vi "TurretAim_OperatorAssist.vi"(0 "Reacquire":bool, 1 "Start":bool, 2 "ManualOverride":bool, 3 "TargetFound":bool, 4 "FullRight":bool, 5 "FullLeft":bool, 8 "TargetPos":dbl format="%#_13g") -> (6 "TurretPos":dbl format="%#_13g", 7 "Current_State":T1=enum."SearchLeft")   [LabVIEW 2016]
uses:
  TypeDefs/TurretAimState_Type.ctl
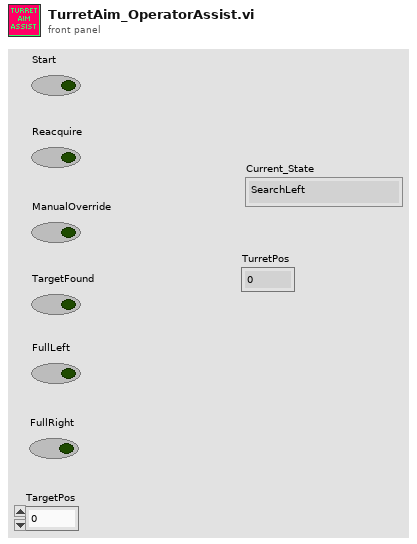
[diagram p1: front panel]
types:
  T1 = typedef "TurretAimState_Type.ctl" = enum16{"Idle", "SearchLeft", "SearchRight", "FindNewTarget", "TargetAcquired"}
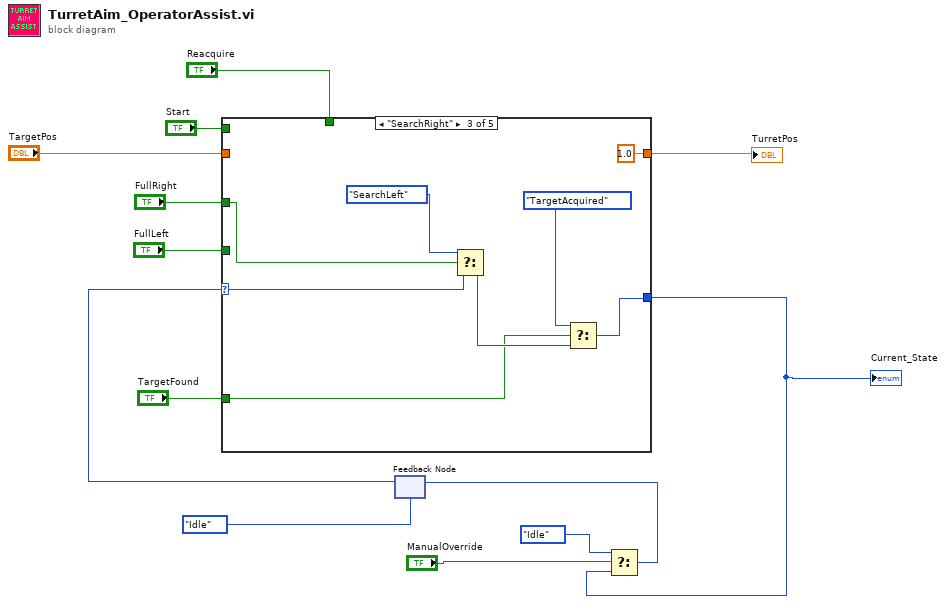
[diagram p0: block diagram]
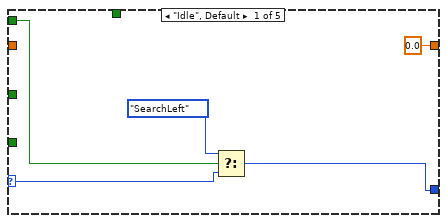
[diagram p2: hidden frame]
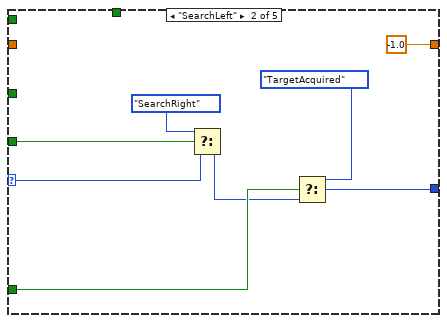
[diagram p3: hidden frame]
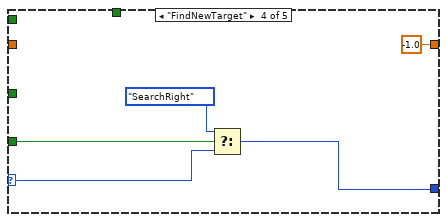
[diagram p4: hidden frame]
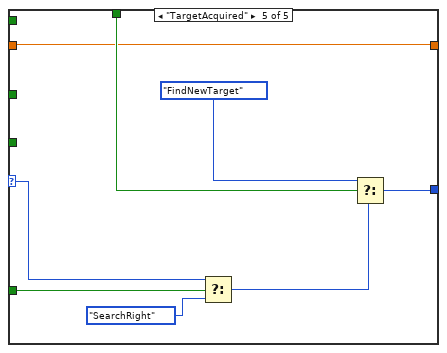
[diagram p5: hidden frame]
diagram:
  n1 = feedback #1(TurretAimState_Type."Idle" ("TurretState")) -> (w13:T1)
  n2 = case shown="\"SearchRight\"" w13 {
    selector: w13 -> [w18 w26 w31 w38 w42]
    tunnel: "TargetFound" -> [_ w24 w32 _ w44]
    tunnel: "FullLeft" -> [_ w19 _ w39 _]
    tunnel: [w15 w22 w29 w36 w45] -> w2
    tunnel: "FullRight" -> [_ _ w27 _ _]
    tunnel: "Reacquire" -> [_ _ _ _ w47]
    tunnel: "Start" -> [w17 _ _ _ _]
    tunnel: [0.0 ("TargetPos") -1.0 ("TurretPos") 1.0 ("TurretPos") -1.0 ("TargetPos") w40] -> w4
    tunnel: "TargetPos" -> [_ _ _ _ w40]
    frame "Idle", Default {
      n3 = Select(t=TurretAimState_Type."SearchLeft", s=w17, f=w18) -> (s? t:f=w15:T1)
    }
    frame "SearchLeft" {
      n4 = Select(t=TurretAimState_Type."SearchRight", s=w19, f=w26) -> (s? t:f=w23:T1)
      n5 = Select(t=TurretAimState_Type."TargetAcquired", s=w24, f=w23) -> (s? t:f=w22:T1)
    }
    frame "SearchRight" {
      n6 = Select(t=TurretAimState_Type."SearchLeft", s=w27, f=w31) -> (s? t:f=w33:T1)
      n7 = Select(t=TurretAimState_Type."TargetAcquired", s=w32, f=w33) -> (s? t:f=w29:T1)
    }
    frame "FindNewTarget" {
      n8 = Select(t=TurretAimState_Type."SearchRight", s=w39, f=w38) -> (s? t:f=w36:T1)
    }
    frame "TargetAcquired" {
      n9 = Select(t=w42, s=w44, f=TurretAimState_Type."SearchRight" ("t")) -> (s? t:f=w43:T1)
      n10 = Select(t=TurretAimState_Type."FindNewTarget", s=w47, f=w43) -> (s? t:f=w45:T1)
    }
  }
  "TurretPos" <- w4
  "Current_State" <- w2
  n11 = Select(t=TurretAimState_Type."Idle", s="ManualOverride", f=w2) -> (s? t:f=w5:T1)
  n12 = feedback-in #1(w5) -> ()
